vi "GUI_CH1_Comm_ZEROMQ.vi"() -> ()   [LabVIEW 2018]
uses:
  RxTx/RxTx.lvclass
  <vilib>/addons/zeromq/socket_type.ctl
  <vilib>/addons/zeromq/zmq_context.lvclass
  <vilib>/addons/zeromq/zeromq.lvlib
  <vilib>/addons/zeromq/zmq_socket.lvclass
panel:
  out "error out":errorcluster
  in  "stop":bool
  out "error out 3":errorcluster
  in  "RxTx.lvclass 2":refnum<class "RxTx.lvclass">
  in  "Channel":u16=1
  # "Channel 1 - TCPIP Communication"
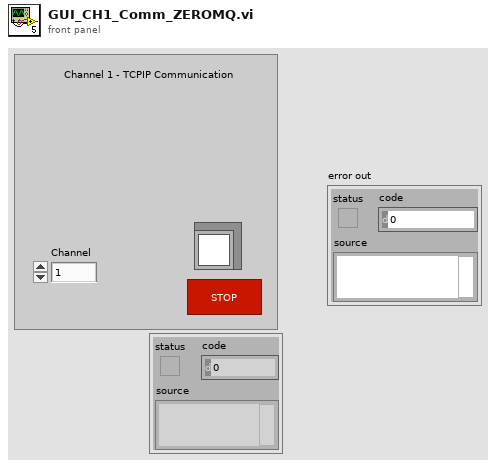
[diagram p1: front panel]
types:
  T1 = typedef "zeromq.lvlib/socket_type.ctl" = enum8{"ZMQ_PAIR", "ZMQ_PUB", "ZMQ_SUB", "ZMQ_REQ", "ZMQ_REP", "ZMQ_DEALER", "ZMQ_ROUTER", "ZMQ_PULL", "ZMQ_PUSH", "ZMQ_XPUB", "ZMQ_XSUB", "ZMQ_STREAM", "ZMQ_SERVER", "ZMQ_CLIENT", "ZMQ_RADIO", "ZMQ_DISH", "ZMQ_GATHER", "ZMQ_SCATTER", "ZMQ_DGRAM"}
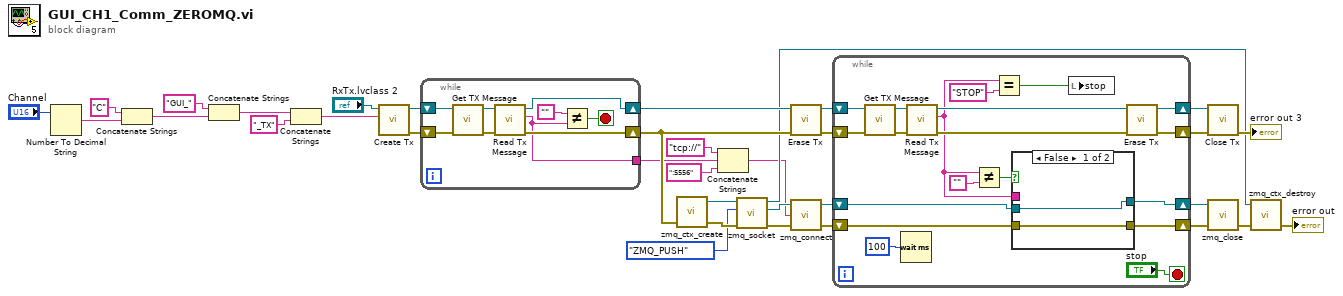
[diagram p0: block diagram]
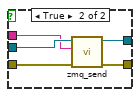
[diagram p2: hidden frame]
diagram:
  n1 = Number To Decimal String(number="Channel") -> (decimal integer string=w33:string)  [unwired: 1 in]
  n2 = Concatenate Strings("C", w33) -> (w23:string)
  n3 = Concatenate Strings("GUI_", w23) -> (w24:string)
  n4 = Concatenate Strings(w24, "_TX" ("Reader Name")) -> (w32:string)
  n5 = call "Create Tx.vi"("Writer Name"=w32, "RxTx in"="RxTx.lvclass 2") -> ("error out"=w18:errorcluster, "RxTx out"=w19:refnum<class "RxTx.lvclass">)  [unwired: 8 in]
  n6 = while {
    shift-right: [w39] -> w9
    shift-left: w18 -> [w38]
    shift-right: [w37] -> w22
    shift-left: w19 -> [w36]
    tunnel: [w35] -> w1
    stop <- w40 stop-if-true
    n7 = call "Get TX Message.vi"("error in (no error)"=w38, "RxTx in"=w36) -> ("error out"=w42:errorcluster, "RxTx out"=w43:refnum<class "RxTx.lvclass">)  [unwired: 8 in]
    n8 = call "Read Tx Message.vi"("error in (no error)"=w42, "RxTx in"=w43) -> ("error out"=w39:errorcluster, "Tx Message"=w35:string, "RxTx out"=w37:refnum<class "RxTx.lvclass">)  [unwired: 7 in]
    n9 = Not Equal?(x="", y=w35) -> (x != y?=w40:bool)
  }
  n10 = call <vilib>:"zmq_ctx_create.vi"("error in"=w9) -> ("error out"=w15:errorcluster, "context out"=w16:refnum<class "zmq_context.lvclass">)  [unwired: 3 in]
  n11 = Concatenate Strings("tcp://" ("endpoint"), w1, ":5556" ("endpoint")) -> (w3:string)
  n12 = call <vilib>:"zmq_socket.vi"("error in"=w15, "socket type"=socket_type."ZMQ_PUSH", "context in"=w16) -> ("error out"=w2:errorcluster, "socket out"=w4:refnum<class "zmq_socket.lvclass">, "context out"=w8:refnum<class "zmq_context.lvclass">)  [unwired: 2 in]
  n13 = call "Erase Tx.vi"("error in (no error)"=w9, "RxTx in"=w22) -> ("error out"=w20:errorcluster, "RxTx out"=w21:refnum<class "RxTx.lvclass">)  [unwired: 8 in]
  n14 = call <vilib>:"zmq_connect.vi"("error in"=w2, "endpoint"=w3, "socket in"=w4) -> ("error out"=w6:errorcluster, "socket out"=w5:refnum<class "zmq_socket.lvclass">)  [unwired: 1 in]
  n15 = while {
    shift-right: [w62] -> w30
    shift-left: w21 -> [w55]
    shift-right: [w61] -> w29
    shift-left: w20 -> [w54]
    shift-right: [w49] -> w12
    shift-left: w6 -> [w50]
    shift-right: [w48] -> w11
    shift-left: w5 -> [w51]
    stop <- "stop" stop-if-true
    n16 = call "Get TX Message.vi"("error in (no error)"=w54, "RxTx in"=w55) -> ("error out"=w60:errorcluster, "RxTx out"=w56:refnum<class "RxTx.lvclass">)  [unwired: 8 in]
    n17 = Wait (ms)(milliseconds to wait=u32 100) -> ()  [unwired: 1 out]
    n18 = call "Read Tx Message.vi"("error in (no error)"=w60, "RxTx in"=w56) -> ("error out"=w57:errorcluster, "Tx Message"=w47:string, "RxTx out"=w58:refnum<class "RxTx.lvclass">)  [unwired: 7 in]
    n19 = Not Equal?(x=w47, y="") -> (x != y?=w44:bool)
    n20 = Equal?(x=w47, y="STOP" ("endpoint")) -> (x = y?=w45:bool)
    n21 = case shown="False" w44 {
      tunnel: w47 -> [_ w65]
      tunnel: w51 -> [w64 w69]
      tunnel: w50 -> [w63 w68]
      tunnel: [w63 w67] -> w49
      tunnel: [w64 w66] -> w48
      frame False {
      }
      frame True {
        n22 = call <vilib>:"zmq_send.vi"("error in"=w68, "data"=w65, "socket in"=w69) -> ("error out"=w67:errorcluster, "socket out"=w66:refnum<class "zmq_socket.lvclass">)  [unwired: 4 in]
      }
    }
    n23 = local write "stop"(w45) -> ()
    n24 = call "Erase Tx.vi"("error in (no error)"=w57, "RxTx in"=w58) -> ("error out"=w61:errorcluster, "RxTx out"=w62:refnum<class "RxTx.lvclass">)  [unwired: 8 in]
  }
  n25 = call "Close Tx.vi"("error in (no error)"=w29, "RxTx in"=w30) -> ("error out"=→"error out 3":errorcluster)  [unwired: 8 in, 1 out]
  n26 = call <vilib>:"zmq_close.vi"("error in"=w12, "socket"=w11) -> ("error out"=w13:errorcluster)  [unwired: 3 in]
  n27 = call <vilib>:"zmq_ctx_destroy.vi"("error in"=w13, "context in"=w8) -> ("error out"=→"error out":errorcluster)  [unwired: 3 in]
